vi "initialize TurnTable Device.vi"(8 "error in (no error)":errorcluster, 10 "VISA resource name":refnum<visa-resource-name>, 11 "AUDIX EM1000 in":refnum<class "AUDIX EM1000.lvclass">) -> (0 "error out":errorcluster, 3 "AUDIX EM1000 out":refnum<class "AUDIX EM1000.lvclass">)   [LabVIEW 2023, in "Turn Table and Mast.lvlib" / "AUDIX EM1000.lvclass"]
uses:
  AUDIX EM1000.lvclass
  AUDIX EM1000.lvclass/AUDIX EM1000.ctl
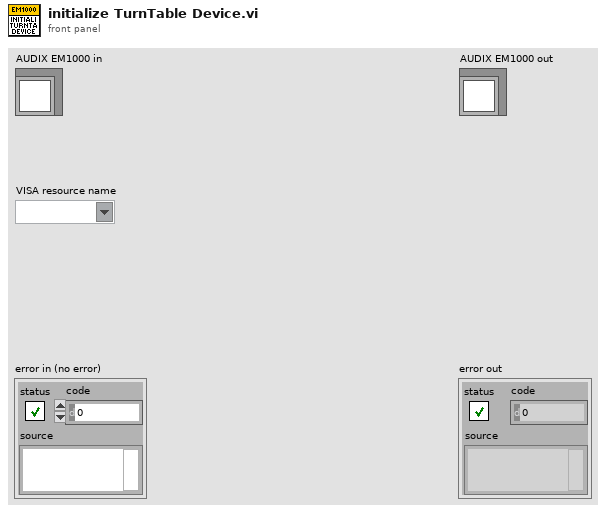
[diagram p1: front panel]
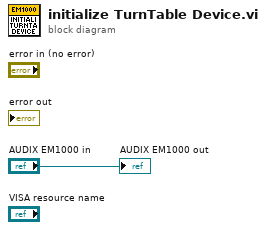
[diagram p0: block diagram]
diagram:
  "AUDIX EM1000 out" <- "AUDIX EM1000 in"
